vi "I2C Read Register (16bit).vi"(7 "MSB(yte) First? (F=Lo->Hi)":bool, 8 "error in (no error)":errorcluster, 10 "Register Address":u8, 11 "LINX I2C in":refnum<class "LINX I2C.lvclass">) -> (0 "error out":errorcluster, 2 "Value":u16, 3 "LINX I2C out":refnum<class "LINX I2C.lvclass">)   [LabVIEW 2020, in "LINX I2C.lvclass"]
doc: "Reads a 16-bit register from the I2C device."
uses:
  LINX I2C.lvclass
panel:
  out "Boolean array":bool[](array[boolean])
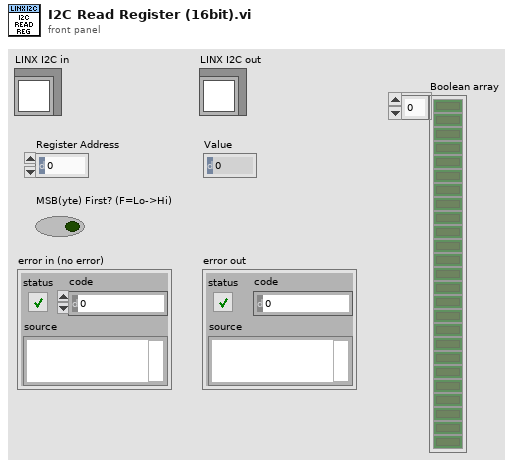
[diagram p1: front panel]
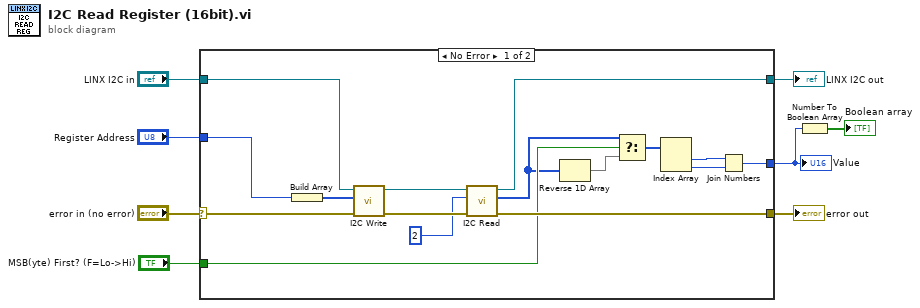
[diagram p0: block diagram]
diagram:
  n1 = case shown="No Error" "error in (no error)" {
    selector: "error in (no error)" -> [w19 w25]
    tunnel: [w17 w26] -> w8
    tunnel: "LINX I2C in" -> [w18 w26]
    tunnel: [w16 w25] -> w6
    tunnel: "Register Address" -> [w20 _]
    tunnel: [w13 _] -> w3
    tunnel: "MSB(yte) First? (F=Lo->Hi)" -> [w12 _]
    frame No Error {
      n2 = Build Array(w20) -> (w22:u8[])
      n3 = call "I2C Write.vi"("error in (no error)"=w19, "Bytes to Write"=w22, "LINX I2C in"=w18) -> ("error out"=w24:errorcluster, "LINX I2C out"=w23:refnum<class "LINX I2C.lvclass">)  [unwired: 7 in]
      n4 = call-dynamic "I2C Read.vi"("error in (no error)"=w24, "# Bytes to Read"=u8 2, "LINX I2C in"=w23) -> ("error out"=w16:errorcluster, "Bytes Read"=w11:u8[], "LINX I2C out"=w17:refnum<class "LINX I2C.lvclass">)  [unwired: 6 in]
      n5 = Reverse 1D Array(array=w11) -> (reversed array=w10:u8[])
      n6 = Select(t=w11, s=w12, f=w10) -> (s? t:f=w9:u8[])
      n7 = Index Array(array=w9) -> (element #1=w15:u8, element #2=w14:u8)  [unwired: 2 in]
      n8 = Join Numbers(hi=w15, lo=w14) -> ((hi.lo)=w13:u16)
    }
    frame Error {
    }
  }
  "LINX I2C out" <- w8
  "error out" <- w6
  "Value" <- w3
  n9 = Number To Boolean Array(number=w3) -> (Boolean array=→"Boolean array":bool[])
